vi "main_test.vi"() -> ()   [LabVIEW 2025]
uses:
  <vilib>/rvi/DesktopExecutionNode/DesktopExecutionNode.xnode
  <vilib>/rvi/DesktopExecutionNode/Execution/niFpgaDEN_Execute.vi
panel:
  in  "Shake forward":bool
  in  "Shake left":bool
  out "Waveform Acc Max":T1(graph)
  out "Waveform Acc Now":T2(graph)
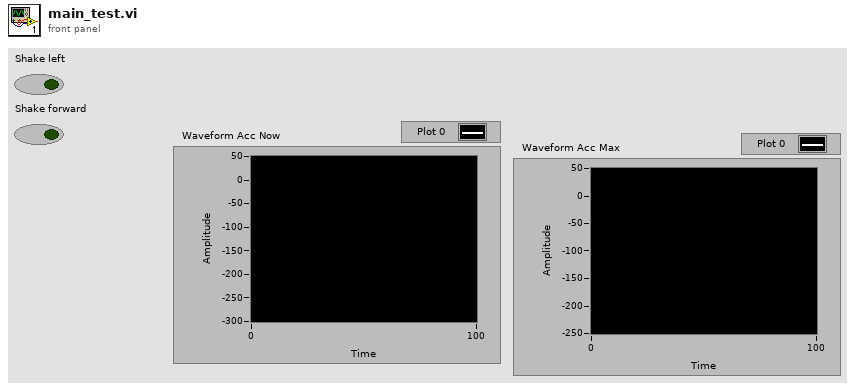
[diagram p1: front panel]
types:
  T1 = cluster{"AccelerationX Max":i16, "AccelerationY Max":i16, "AccelerationZ Max":i16}
  T2 = cluster{"AccelerationX Now":i16, "AccelerationY Now":i16, "AccelerationZ Now":i16}
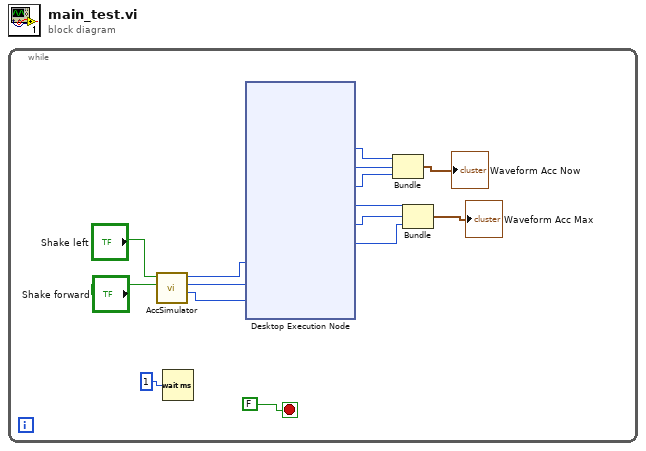
[diagram p0: block diagram]
diagram:
  n1 = while {
    stop <- FALSE stop-if-true
    n2 = call "AccSimulator.vi"("Shake forward"="Shake forward", "Shake left"="Shake left") -> ("Acc Y"=w11:i16, "Acc X"=w12:i16, "Acc Z"=w13:i16)  [unwired: 7 in]
    n3 = Wait (ms)(milliseconds to wait=u32 1) -> ()  [unwired: 1 out]
    n4 = xnode "Desktop Execution Node"("AccelerationZ"=w13, "AccelerationX"=w12, "AccelerationY"=w11) -> ("AccelerationX Now"=w10:i16, "AccelerationY Now"=w9:i16, "AccelerationZ Now"=w8:i16, "AccelerationX Max"=w6:i16, "AccelerationY Max"=w5:i16, "AccelerationZ Max"=w4:i16)  [unwired: 1 in, 1 out]
    n5 = Bundle("AccelerationX Now"=w10, "AccelerationY Now"=w9, "AccelerationZ Now"=w8) -> (→"Waveform Acc Now":T2)  [unwired: 1 in]
    n6 = Bundle("AccelerationX Max"=w6, "AccelerationY Max"=w5, "AccelerationZ Max"=w4) -> (→"Waveform Acc Max":T1)  [unwired: 1 in]
  }
